vi "_Match String Inside Pattern.vi"(7 "Cluster":cluster{"left":string, "right":string}={"left"="(", "right"=")"}, 11 "string":string) -> (2 "Keys":string[](array[string]), 3 "String inside":string)   [LabVIEW 2017, in "csmdoc.lvlib"]
uses:
  csmdoc.lvlib
  _Shared/CSM Shared.lvlib
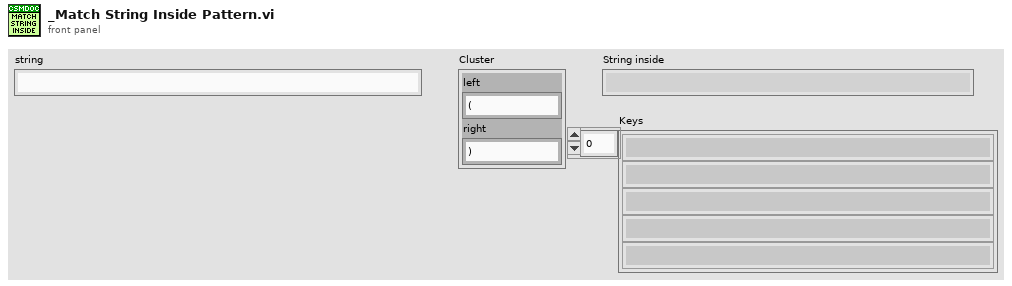
[diagram p1: front panel]
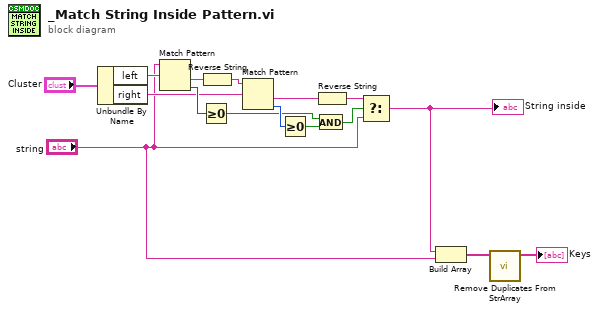
[diagram p0: block diagram]
diagram:
  n1 = Unbundle By Name("Cluster") -> ("left"=w9:string, "right"=w8:string)
  n2 = Match Pattern(string="string", regular expression=w9) -> (after substring=w16:string, offset past match=w14:i32)  [unwired: 1 in, 2 out]
  n3 = Greater Or Equal To 0?(x=w14) -> (x >= 0?=w13:bool)
  n4 = Reverse String(1:w16) -> (0:w7:string)
  n5 = Match Pattern(string=w7, regular expression=w8) -> (after substring=w6:string, offset past match=w15:i32)  [unwired: 1 in, 2 out]
  n6 = Greater Or Equal To 0?(x=w15) -> (x >= 0?=w12:bool)
  n7 = And(x=w13, y=w12) -> (x .and. y?=w11:bool)
  n8 = Reverse String(1:w6) -> (0:w5:string)
  n9 = Select(t=w5, s=w11, f="string") -> (s? t:f=w3:string)
  "String inside" <- w3
  n10 = Build Array(w3, "string") -> (w4:string[])
  n11 = call "Remove Duplicates From StrArray.vi"("StrArray In"=w4) -> ("StrArray"=→"Keys":string[])  [unwired: 9 in, 1 out]
